vi "Probe_Add.vi"(0 "a":dbl, 1 "b":dbl) -> (4 "sum":dbl)   [LabVIEW 2026]
doc: "LabVIEW 2019 MCP compatibility probe: sum = a + b. Disposable."
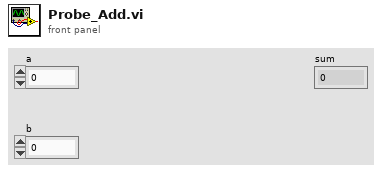
[diagram p1: front panel]
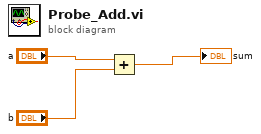
[diagram p0: block diagram]
diagram:
  n1 = Add(x="a", y="b") -> (x+y=→"sum":dbl)
